vi "Create Error Cluster from Response Body.vi"(7 "AWS Core":refnum<class "HTTP Request.lvclass">, 8 "error in (no error)":errorcluster, 11 "Response body":string) -> (0 "error out":errorcluster, 3 "Is Throttled?":bool)   [LabVIEW 2015, in "NI_AWS_Core.lvlib" / "HTTP Request.lvclass"]
uses:
  HTTP Request.lvclass
  XML Parsing/NI_XML Parsing.lvlib
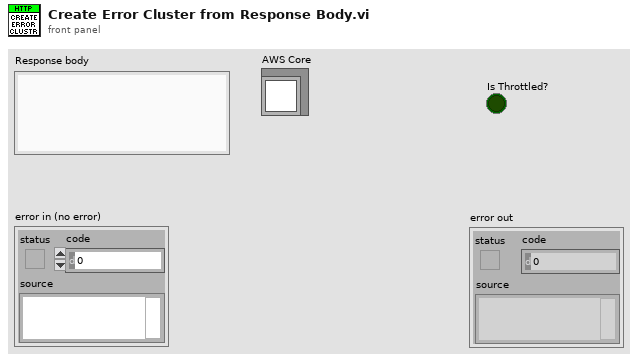
[diagram p1: front panel]
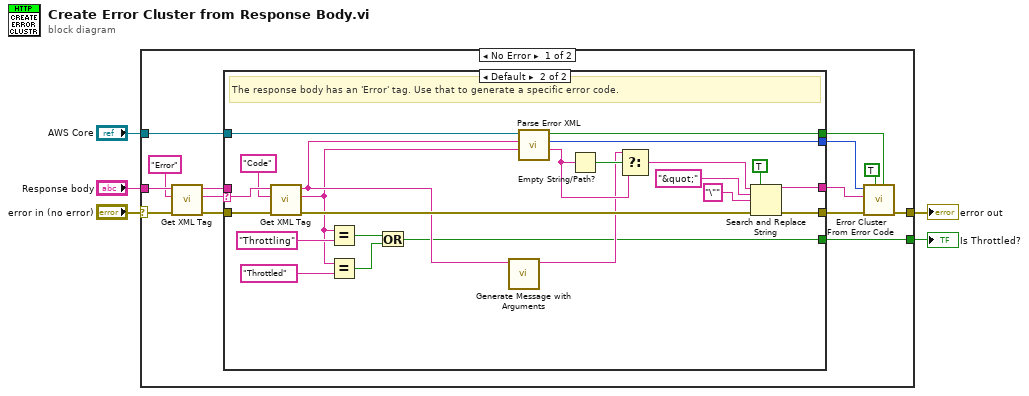
[diagram p0: block diagram]
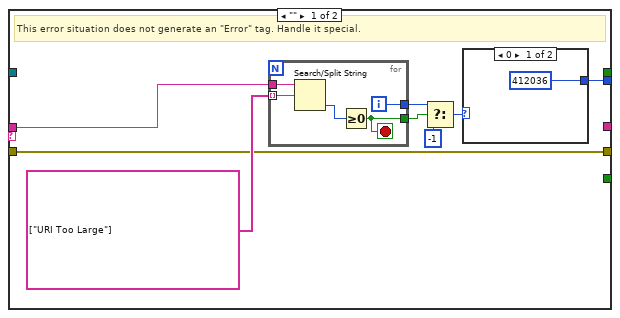
[diagram p2: hidden frame]
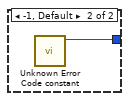
[diagram p3: hidden frame]
diagram:
  n1 = case shown="No Error" "error in (no error)" {
    selector: "error in (no error)" -> [w15 w58]
    tunnel: "Response body" -> [w19 _]
    tunnel: [w14 w58] -> w4
    tunnel: [w12 _] -> w2
    tunnel: "AWS Core" -> [w11 _]
    frame No Error {
      n2 = call "Get XML Tag.vi"("error in (no error)"=w15, "Tag name"="Error", "XML String in"=w19) -> ("error out"=w17:errorcluster, "Tag value"=w16:string, "XML String dup"=w6:string)  [unwired: 4 in, 2 out]
      n3 = case shown="Default" w16 {
        selector: w16 -> [_ w56]
        tunnel: w17 -> [w26 w57]
        tunnel: [_ w36] -> w12
        tunnel: w11 -> [_ w52]
        tunnel: [_ w51] -> w10
        tunnel: [w25 w50] -> w9
        tunnel: [w26 w46] -> w8
        tunnel: [_ w44] -> w7
        tunnel: w6 -> [w20 _]
        frame "" {
          # "This error situation does not generate an \"Error\" tag. Handle it special."
          n4 = for {
            tunnel: string[] ["URI Too Large"] -> [w30] mode=indexing
            tunnel: [w28] -> w24
            tunnel: [w31] -> w23
            tunnel: w20 -> [w29]
            i -> [w28]
            stop <- w31 stop-if-true
            n5 = Search/Split String(string=w29, search string/char (-)=w30) -> (offset of match=w32:i32)  [unwired: 1 in, 2 out]
            n6 = Greater Or Equal To 0?(x=w32) -> (x >= 0?=w31:bool)
          }
          n7 = Select(t=w24, s=w23, f=-1) -> (s? t:f=w22:i32)
          n8 = case shown="0" w22 {
            tunnel: [412036 w34] -> w25
            frame 0 {
            }
            frame -1, Default {
              n9 = call "Unknown Error Code constant.vi"() -> ("AWS Unknown Error Code value"=w34:i32)  [unwired: 11 in]
            }
          }
        }
        frame Default {
          # "The response body has an 'Error' tag. Use that to generate a specific error code."
          n10 = call "Get XML Tag.vi"("error in (no error)"=w57, "Tag name"="Code", "XML String in"=w56) -> ("error out"=w47:errorcluster, "Tag value"=w37:string, "XML String dup"=w43:string)  [unwired: 4 in, 2 out]
          n11 = Equal?(x=w37, y="Throttling") -> (x = y?=w53:bool)
          n12 = Equal?(x=w37, y="Throttled") -> (x = y?=w35:bool)
          n13 = Or(x=w53, y=w35) -> (x .or. y?=w36:bool)
          n14 = call "Generate Message with Arguments.vi"("XML String"=w43) -> ("Message with Arguments"=w39:string)  [unwired: 10 in]
          n15 = call-dynamic "Parse Error XML.vi"("Code Tag Value"=w37, "Error XML"=w43, "AWS Core"=w52) -> ("Error Description Override"=w41:string, "Error Code"=w50:i32, "Warning"=w51:bool)  [unwired: 6 in]
          n16 = Empty String/Path?(string/path=w41) -> (empty?=w42:bool)
          n17 = Select(t=w39, s=w42, f=w41) -> (s? t:f=w40:string)
          n18 = Search and Replace String(replace all?=TRUE ("replace all? (F)"), input string=w40, search string="&quot;", replace string="\"", error in=w47) -> (result string=w44:string, error out=w46:errorcluster)  [unwired: 3 in, 2 out]
        }
      }
      n19 = call <vilib>:"Error Cluster From Error Code.vi"("is warning? (False)"=w10, "show call chain? (False)"=TRUE, "error in (no error)"=w8, "error message (\"\")"=w7, "error code (0)"=w9) -> ("error out"=w14:errorcluster)  [unwired: 4 in]
    }
    frame Error {
    }
  }
  "error out" <- w4
  "Is Throttled?" <- w2
